vi "Update WebView2 Assembly.vi"   [LabVIEW 2020]
uses:
  WebView2 Updater/WebView2 Updater.vi
  WebView2 Updater/WebView2 Updater.lvclass
types:
  T1 = enum32{"Invalid", "Standard", "Closed", "Hidden", "Minimized", "Maximized"}
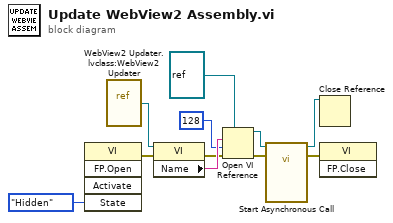
[diagram p0: block diagram]
diagram:
  n1 = invoke class="VI" method="FP.Open"("State"=T1."Hidden") -> (error out=w4:errorcluster)  [unwired: 4 in, 4 out]
  n2 = vi-ref "WebView2 Updater.lvclass:WebView2 Updater.vi"() -> (w10:refnum<vi>)
  n3 = property class="VI"(reference=w10, error in=w4) -> (error out=w6:errorcluster, "Name"=w9:string)  [unwired: 1 out]
  n4 = Open VI Reference(type specifier VI Refnum (for type only)=refnum<vi> refnum ("reference out"), vi path=w9, options=128, error in (no error)=w6) -> (vi reference=w7:refnum<vi>, error out=w5:errorcluster)  [unwired: 2 in]
  n5 = call-by-ref "Start Asynchronous Call"(reference=w7, error in=w5) -> (reference out=w2:refnum<vi>, error out=w1:errorcluster)  [unwired: 12 in]
  n6 = Close Reference(reference=w2) -> ()  [unwired: 1 in, 1 out]
  n7 = invoke class="VI" method="FP.Close"(error in=w1) -> ()  [unwired: 2 in, 3 out]
